vi "Launch Nested Actors.vi"(8 "error in (no error)":errorcluster, 10 "Selection UI Subpanel Ref":refnum<vi>, 11 "Pane Relief Main UI in":refnum<class "Pane Relief Main UI.lvclass">) -> (0 "error out":errorcluster, 3 "Pane Relief Main UI out":refnum<class "Pane Relief Main UI.lvclass">)   [LabVIEW 2015, in "Pane Relief Main UI.lvlib" / "Pane Relief Main UI.lvclass"]
uses:
  Pane Relief Main UI.lvclass
  Splitter Settings UI/Splitter Settings UI/Splitter Settings UI.lvclass
  Instructions UI/Instructions UI/Instructions UI.lvclass
  Panel Object Actions UI/Panel Object Actions UI/Panel Object Actions UI.lvclass
  Pane Settings UI/Pane Settings UI/Pane Settings UI.lvclass
  Pane Relief Main UI.lvclass/Pane Relief Main UI.ctl
  <vilib>/MGI/Panel Manager/Panel/Panel/Subpanel/Subpanel.vi
  <vilib>/MGI/Panel Manager/Panel Actor/Panel Actor/Panel Actor.lvclass
  <vilib>/MGI/Panel Manager/Panel/Panel.lvlib
  <vilib>/MGI/Panel Manager/Panel/Panel/Subpanel/Subpanel.lvclass
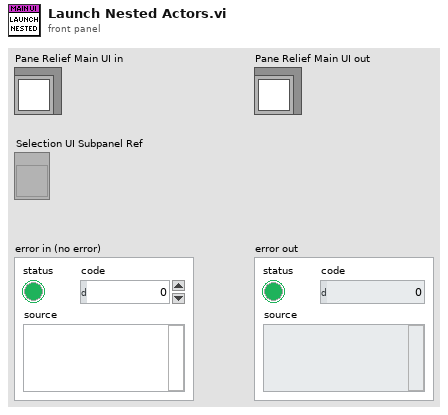
[diagram p1: front panel]
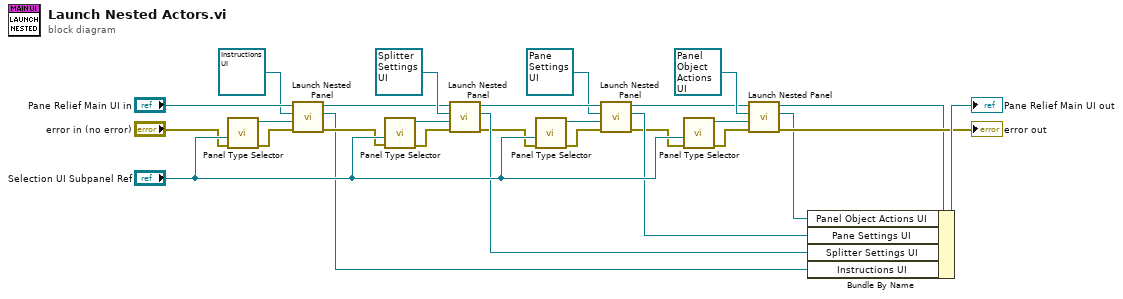
[diagram p0: block diagram]
diagram:
  n1 = call-poly <vilib>:"Panel Type Selector.vi"("Error In"="error in (no error)", "Sub Panel"="Selection UI Subpanel Ref") -> ("Error Out"=w13:errorcluster, "Subpanel Out"=w14:refnum<class "Subpanel.lvclass">)  [unwired: 8 in]
  n2 = call <vilib>:"Launch Nested Panel.vi"("error in (no error)"=w13, "Panel"=w14, "Nested Panel Actor"=refnum<class "Instructions UI.lvclass"> refnum ("Instructions UI.lvlib:Instructions UI.lvclass"), "Panel Actor in"="Pane Relief Main UI in") -> ("error out"=w11:errorcluster, "Nested Actor's Enqueuer"=w9:refnum<class "Message Enqueuer.lvclass">, "Panel Actor out"=w10:refnum<class "Pane Relief Main UI.lvclass">)  [unwired: 4 in, 1 out]
  n3 = call-poly <vilib>:"Panel Type Selector.vi"("Error In"=w11, "Sub Panel"="Selection UI Subpanel Ref") -> ("Error Out"=w18:errorcluster, "Subpanel Out"=w17:refnum<class "Subpanel.lvclass">)  [unwired: 8 in]
  n4 = call <vilib>:"Launch Nested Panel.vi"("error in (no error)"=w18, "Panel"=w17, "Nested Panel Actor"=refnum<class "Splitter Settings UI.lvclass"> refnum ("Splitter Settings UI.lvlib:Splitter Settings UI.lvclass"), "Panel Actor in"=w10) -> ("error out"=w21:errorcluster, "Nested Actor's Enqueuer"=w23:refnum<class "Message Enqueuer.lvclass">, "Panel Actor out"=w20:refnum<class "Pane Relief Main UI.lvclass">)  [unwired: 4 in, 1 out]
  n5 = call-poly <vilib>:"Panel Type Selector.vi"("Error In"=w21, "Sub Panel"="Selection UI Subpanel Ref") -> ("Error Out"=w2:errorcluster, "Subpanel Out"=w3:refnum<class "Subpanel.lvclass">)  [unwired: 8 in]
  n6 = call <vilib>:"Launch Nested Panel.vi"("error in (no error)"=w2, "Panel"=w3, "Nested Panel Actor"=refnum<class "Pane Settings UI.lvclass"> refnum ("Pane Settings UI.lvlib:Pane Settings UI.lvclass"), "Panel Actor in"=w20) -> ("error out"=w5:errorcluster, "Nested Actor's Enqueuer"=w22:refnum<class "Message Enqueuer.lvclass">, "Panel Actor out"=w4:refnum<class "Pane Relief Main UI.lvclass">)  [unwired: 4 in, 1 out]
  n7 = call-poly <vilib>:"Panel Type Selector.vi"("Error In"=w5, "Sub Panel"="Selection UI Subpanel Ref") -> ("Error Out"=w7:errorcluster, "Subpanel Out"=w6:refnum<class "Subpanel.lvclass">)  [unwired: 8 in]
  n8 = call <vilib>:"Launch Nested Panel.vi"("error in (no error)"=w7, "Panel"=w6, "Nested Panel Actor"=refnum<class "Panel Object Actions UI.lvclass"> refnum ("Panel Object Actions UI.lvlib:Panel Object Actions UI.lvclass"), "Panel Actor in"=w4) -> ("error out"=→"error out":errorcluster, "Nested Actor's Enqueuer"=w15:refnum<class "Message Enqueuer.lvclass">, "Panel Actor out"=w16:refnum<class "Pane Relief Main UI.lvclass">)  [unwired: 4 in, 1 out]
  n9 = Bundle By Name(cluster=w16, "Panel Object Actions UI"=w15, "Pane Settings UI"=w22, "Splitter Settings UI"=w23, "Instructions UI"=w9) -> (→"Pane Relief Main UI out":refnum<class "Pane Relief Main UI.lvclass">)
